vi "SPARK Open Brushless.vi"(8 "error in":errorcluster, 10 "deviceId":i32, 11 "busID":i32) -> (0 "error out":errorcluster, 3 "Spark refnum":T2)   [LabVIEW 2023, in "REVLibDriver.lvlib"]
uses:
  <vilib>/REVLibDriver/REVLibDriver.lvlib
  <vilib>/REV Custom Controls/REVSparkRefnum.ctl
  <vilib>/REVLibDriver/subvi/RevLibError.ctl
  <vilib>/REV Custom Controls/c_Spark_SparkModel.ctl
  <vilib>/REV Custom Controls/c_Spark_MotorType.ctl
  REVLibDriver.so
panel:
  out "status out":T1
  out "function return":T1
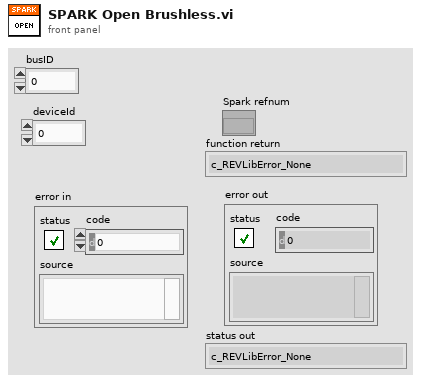
[diagram p1: front panel]
types:
  T1 = typedef "REVLibDriver.lvlib/RevLibError.ctl" = enum16{"c_REVLibError_None", "c_REVLibError_General", "c_REVLibError_CANTimeout", "c_REVLibError_NotImplemented", "c_REVLibError_HAL", "c_REVLibError_CantFindFirmware", "c_REVLibError_FirmwareTooOld", "c_REVLibError_FirmwareTooNew", "c_REVLibError_ParamInvalidID", "c_REVLibError_ParamMismatchType", "c_REVLibError_ParamAccessMode", "c_REVLibError_ParamInvalid", "c_REVLibError_ParamNotImplementedDeprecated", "c_REVLibError_FollowConfigMismatch", "c_REVLibError_Invalid", "c_REVLibError_SetpointOutOfRange", "c_REVLibError_Unknown", "c_REVLibError_CANDisconnected", "c_REVLibError_DuplicateCANId", "c_REVLibError_InvalidCANId", "c_REVLibError_SparkMaxDataPortAlreadyConfiguredDifferently", "c_REVLibError_SparkFlexBrushedWithoutDock", "c_REVLibError_InvalidBrushlessEncoderConfiguration", "c_REVLibError_FeedbackSensorIncompatibleWithDataPortConfig", "c_REVLibError_ParamInvalidChannel", "c_REVLibError_ParamInvalidValue", "c_REVLibError_CannotPersistParametersWhileEnabled", "c_REVLibError_NotReadyToReceiveCommand", "c_REVLibError_NumCodes"}
  T2 = typedef "REVLibDriver.lvlib/REVSparkRefnum.ctl" = refnum<k20>
  T3 = typedef "REVLibDriver.lvlib/c_Spark_MotorType.ctl" = enum16{"c_Spark_kMotorType_BRUSHED", "    c_Spark_kMotorType_BRUSHLESS", "    c_Spark_kNumMotorTypes"}
  T4 = typedef "REVLibDriver.lvlib/c_Spark_SparkModel.ctl" = u16
  T5 = typedef "REVLibDriver.lvlib/c_Spark_handle.ctl" = cluster{"Pointer":u64}
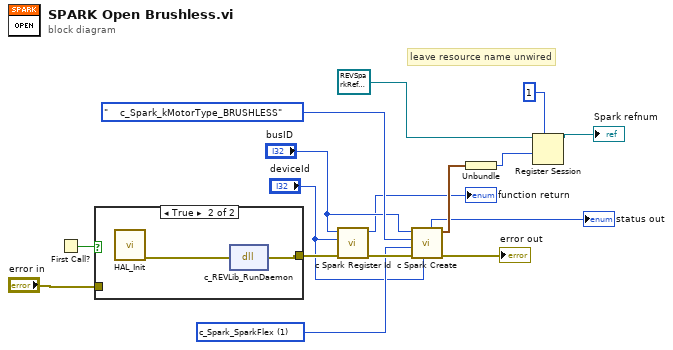
[diagram p0: block diagram]
diagram:
  w15 = T4 1 items=["c_Spark_SparkMax"=0, "c_Spark_SparkFlex"=1, "c_Spark_Unknown"=255] ("unconfirmedModel")
  # "leave resource name unwired"
  n1 = First Call?() -> (First Call?: T/F=w11:bool)
  n2 = case shown="True" w11 {
    tunnel: [w17 w19] -> w13
    tunnel: "error in" -> [w17 _]
    frame False {
    }
    frame True {
      n3 = call <vilib>:"HAL_Init.vi"() -> ("error out"=w18:errorcluster)  [unwired: 11 in]
      n4 = dll-call lib="REVLibDriver.*" fn="c_REVLib_RunDaemon"(error in=w18) -> (error out=w19:errorcluster)  [unwired: 3 in, 1 out]
    }
  }
  n5 = call <vilib>:"c Spark Register Id.vi"("error in (no error)"=w13, "deviceId"="deviceId", "busID"="busID") -> ("error out"=w16:errorcluster, "function return"=→"function return":T1)  [unwired: 7 in]
  n6 = call <vilib>:"c Spark Create.vi"("deviceId"="deviceId", "error in (no error)"=w16, "unconfirmedModel"=w15, "type"=c_Spark_MotorType."    c_Spark_kMotorType_BRUSHLESS", "busId"="busID") -> ("error out"=→"error out":errorcluster, "handle"=w7:T5, "status out"=→"status out":T1)  [unwired: 4 in]
  n7 = Unbundle(w7) -> ("Pointer"=w6:u64)
  n8 = Register Session(7:1 ("cleanup mode (default to class = 0)"), 9:w6, 11:T2 refnum ("REV Spark Refnum")) -> (3:→"Spark refnum":T2)  [unwired: 2 in, 1 out]
